vi "VIH Utility - UI - Get Underlined Substring at Offset (String Control).vi"(6 "Get string (T)":bool=TRUE, 8 "error in":errorcluster, 10 "Offset":i32, 11 "Str Refnum":refnum<vi>) -> (0 "error out":errorcluster, 1 "Selection":cluster{"Start":i32, "End":i32}, 2 "String":string, 3 "dup Str Refnum":refnum<vi>, 4 "active":bool)   [LabVIEW 2014]
doc: "::: VI Helpeks :::\nCopyright (c) 2000-2026 Konstantin Shifershteyn. All rights reserved."
panel:
  # "VI Helpeks\nCopyright (c) 2012-2026 Konstantin Shifershteyn"
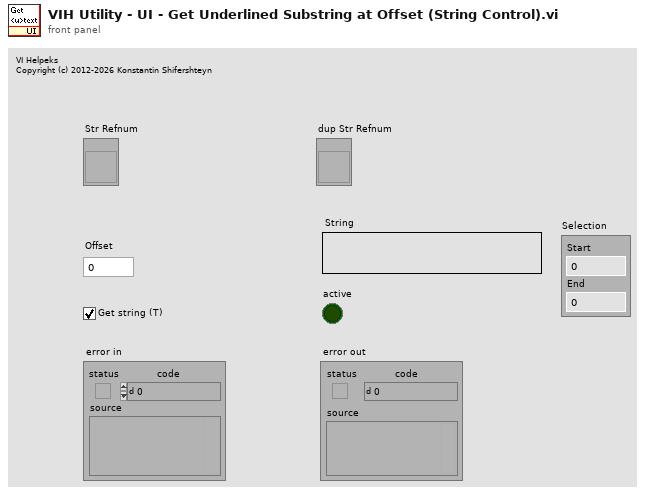
[diagram p1: front panel]
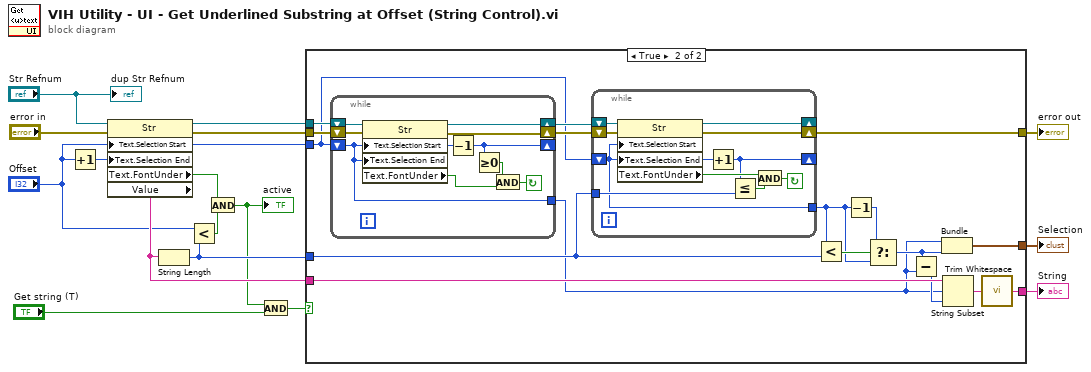
[diagram p0: block diagram]
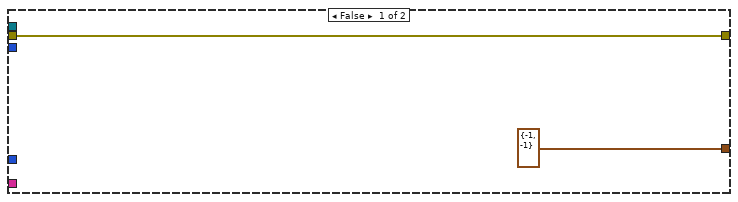
[diagram p2: hidden frame]
diagram:
  n1 = Increment(x="Offset") -> (x+1=w14:i32)
  n2 = property class="Str"(reference="Str Refnum", error in="error in", "Text.Selection Start"="Offset", "Text.Selection End"=w14) -> (reference out=w16:refnum<vi>, error out=w13:errorcluster, "Text.FontUnder"=w8:bool, "Value"=w10:string)
  n3 = String Length(string=w10) -> (length=w5:i32)
  n4 = Less?(x="Offset", y=w5) -> (x < y?=w7:bool)
  n5 = And(x=w8, y=w7) -> (x .and. y?=w1:bool)
  "active" <- w1
  n6 = And(x=w1, y="Get string (T)") -> (x .and. y?=w3:bool)
  n7 = case shown="True" w3 {
    tunnel: w16 -> [_ w35]
    tunnel: "Offset" -> [_ w26]
    tunnel: w10 -> [_ w33]
    tunnel: [_ w30] -> w15
    tunnel: w13 -> [w18 w29]
    tunnel: [w18 w27] -> w11
    tunnel: w5 -> [_ w25]
    tunnel: [cluster{"Offest":i32, "Offest":i32} {"Offest"=-1, "Offest"=-1} w19] -> w4
    frame False {
    }
    frame True {
      n8 = while {
        shift-right: [w42] -> _
        shift-left: w26 -> [w36]
        shift-right: [w39] -> w34
        shift-left: w35 -> [w43]
        tunnel: [w36] -> w20
        shift-right: [w37] -> w28
        shift-left: w29 -> [w38]
        stop <- w44 continue-if-true
        n9 = property class="Str"(reference=w43, error in=w38, "Text.Selection Start"=w36, "Text.Selection End"=w36) -> (reference out=w39:refnum<vi>, error out=w37:errorcluster, "Text.FontUnder"=w40:bool)
        n10 = Decrement(x=w36) -> (x-1=w42:i32)
        n11 = Greater Or Equal To 0?(x=w42) -> (x >= 0?=w41:bool)
        n12 = And(x=w41, y=w40) -> (x .and. y?=w44:bool)
      }
      n13 = while {
        shift-right: [w50] -> _
        shift-left: w26 -> [w45]
        tunnel: w25 -> [w51]
        tunnel: [w45] -> w22
        shift-right: [w48] -> _
        shift-left: w34 -> [w52]
        shift-right: [w46] -> w27
        shift-left: w28 -> [w47]
        stop <- w53 continue-if-true
        n14 = property class="Str"(reference=w52, error in=w47, "Text.Selection Start"=w45, "Text.Selection End"=w45) -> (reference out=w48:refnum<vi>, error out=w46:errorcluster, "Text.FontUnder"=w54:bool)
        n15 = Increment(x=w45) -> (x+1=w50:i32)
        n16 = Less Or Equal?(x=w50, y=w51) -> (x <= y?=w49:bool)
        n17 = And(x=w54, y=w49) -> (x .and. y?=w53:bool)
      }
      n18 = Less?(x=w22, y=w25) -> (x < y?=w23:bool)
      n19 = Decrement(x=w22) -> (x-1=w24:i32)
      n20 = Select(t=w24, s=w23, f=w22) -> (s? t:f=w21:i32)
      n21 = Subtract(x=w21, y=w20) -> (x-y=w32:i32)
      n22 = Bundle("Offset"=w20, "Offset"=w21) -> (w19:cluster{"Offset":i32, "Offset":i32})  [unwired: 1 in]
      n23 = String Subset(string=w33, offset (0)=w20, length (rest)=w32) -> (substring=w31:string)
      n24 = call <vilib>:"Trim Whitespace.vi"("string"=w31) -> ("trimmed string"=w30:string)  [unwired: 1 in]
    }
  }
  "String" <- w15
  "error out" <- w11
  "Selection" <- w4
  "dup Str Refnum" <- "Str Refnum"
